vi "FuncVI-Log.vi"(5 "InstanceRef":T2, 9 "arg list":T1[](array[typedef]) {"num" format="%.2f"}) -> (0 "error out":bool, 3 "result":T1 {"num" format="%.2f"})   [LabVIEW 2021]
doc: "::: CalcExpress Toolkit :::\nCopyright (c) 2000-2026 Konstantin Shifershteyn. All rights reserved."
uses:
  cetypes.llb/CalcExpress Function Argument Info.ctl
  cetypes.llb/CalcExpress Instance RefNum.ctl
panel:
  in  "max arg num":i32=2
  in  "min arg num":i32=2
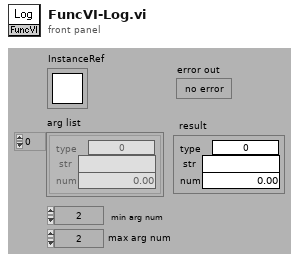
[diagram p1: front panel]
types:
  T1 = typedef "CalcExpress Function Argument Info.ctl" = cluster{"type":u32, "str":string, "num":dbl}
  T2 = typedef "CalcExpress Instance RefNum.ctl" = refnum<k1>
  T3 = enum16{"Array-Array", "Array-Scalar", "Scalar-Array", "Scalar-Scalar"}
  T4 = cluster{"Left 2D":cdb[][], "Left Scalar":cdb, "Right 2D":cdb[][], "Right Scalar":cdb}
  T5 = cluster{"Left 2D":dbl[][], "Left Scalar":dbl, "Right 2D":dbl[][], "Right Scalar":dbl}
  T6 = typedef "CalcExpress Data Type.ctl" = enum32{"String", "DBL Number", "identifier", "1D Array of DBL", "2D Array of DBL", "CDB Number", "1D Array of CDB", "2D Array of CDB", "1D Array of String", "2D Array of String", "Unknown data type"}
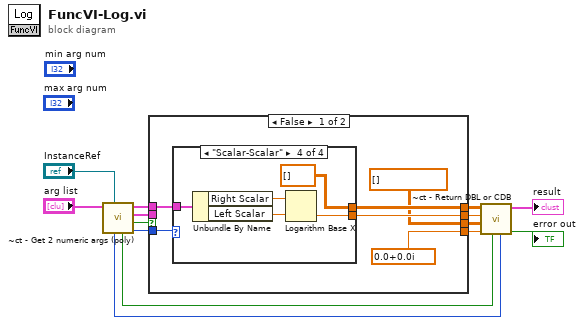
[diagram p0: block diagram]
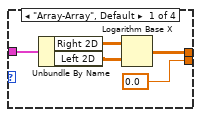
[diagram p2: hidden frame]
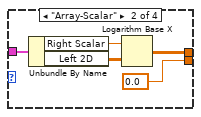
[diagram p3: hidden frame]
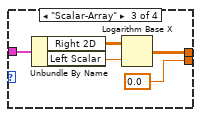
[diagram p4: hidden frame]
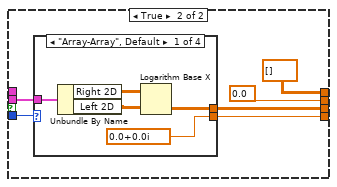
[diagram p5: hidden frame]
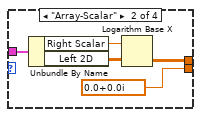
[diagram p6: hidden frame]
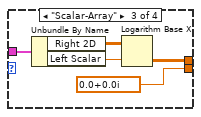
[diagram p7: hidden frame]
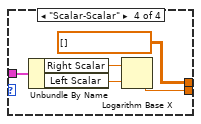
[diagram p8: hidden frame]
diagram:
  n1 = call "~ct - Get 2 numeric args (poly).vi"("InstanceRef"="InstanceRef", "args list"="arg list") -> ("poly"=w5:T3, "CDB ?"=w8:bool, "CDB arguments"=w6:T4, "DBL arguments"=w7:T5, "error out"=w10:bool, "type of result"=w9:T6)  [unwired: 4 in]
  n2 = case shown="False" w8 {
    tunnel: w7 -> [w19 _]
    tunnel: w6 -> [_ w45]
    tunnel: w5 -> [w20 w46]
    tunnel: [w18 dbl[][] []] -> w4
    tunnel: [w17 0.0] -> w3
    tunnel: [cdb[][] [] w44] -> w2
    tunnel: [cdb 0.0+0.0i w43] -> w1
    frame False {
      n3 = case shown="\"Scalar-Scalar\"" w20 {
        tunnel: w19 -> [w25 w30 w35 w40]
        tunnel: [w22 w27 w32 dbl[][] []] -> w18
        tunnel: [0.0 0.0 0.0 w37] -> w17
        frame "Array-Array", Default {
          n4 = Unbundle By Name(w25) -> ("Right 2D"=w24:dbl[][], "Left 2D"=w23:dbl[][])
          n5 = Logarithm Base X(1:w23, 2:w24) -> (0:w22:dbl[][])
        }
        frame "Array-Scalar" {
          n6 = Unbundle By Name(w30) -> ("Right Scalar"=w29:dbl, "Left 2D"=w28:dbl[][])
          n7 = Logarithm Base X(1:w28, 2:w29) -> (0:w27:dbl[][])
        }
        frame "Scalar-Array" {
          n8 = Unbundle By Name(w35) -> ("Right 2D"=w34:dbl[][], "Left Scalar"=w33:dbl)
          n9 = Logarithm Base X(1:w33, 2:w34) -> (0:w32:dbl[][])
        }
        frame "Scalar-Scalar" {
          n10 = Unbundle By Name(w40) -> ("Right Scalar"=w39:dbl, "Left Scalar"=w38:dbl)
          n11 = Logarithm Base X(1:w38, 2:w39) -> (0:w37:dbl)
        }
      }
    }
    frame True {
      n12 = case shown="\"Array-Array\", Default" w46 {
        tunnel: w45 -> [w51 w56 w61 w66]
        tunnel: [w48 w53 w58 cdb[][] []] -> w44
        tunnel: [cdb 0.0+0.0i cdb 0.0+0.0i cdb 0.0+0.0i w63] -> w43
        frame "Array-Array", Default {
          n13 = Unbundle By Name(w51) -> ("Right 2D"=w50:cdb[][], "Left 2D"=w49:cdb[][])
          n14 = Logarithm Base X(1:w49, 2:w50) -> (0:w48:cdb[][])
        }
        frame "Array-Scalar" {
          n15 = Unbundle By Name(w56) -> ("Right Scalar"=w55:cdb, "Left 2D"=w54:cdb[][])
          n16 = Logarithm Base X(1:w54, 2:w55) -> (0:w53:cdb[][])
        }
        frame "Scalar-Array" {
          n17 = Unbundle By Name(w61) -> ("Right 2D"=w60:cdb[][], "Left Scalar"=w59:cdb)
          n18 = Logarithm Base X(1:w59, 2:w60) -> (0:w58:cdb[][])
        }
        frame "Scalar-Scalar" {
          n19 = Unbundle By Name(w66) -> ("Right Scalar"=w65:cdb, "Left Scalar"=w64:cdb)
          n20 = Logarithm Base X(1:w64, 2:w65) -> (0:w63:cdb)
        }
      }
    }
  }
  n21 = call "~ct - Return DBL or CDB.vi"("type"=w9, "error in"=w10, "CDB"=w1, "2D CDB"=w2, "DBL"=w3, "2D DBL"=w4) -> ("error out"=→"error out":bool, "result"=→"result":T1)  [unwired: 4 in]
